vi "Main.vi"(8 "error in":errorcluster, 10 "User Events":T1, 11 "Message Queues in":T2) -> (0 "error out":errorcluster)   [LabVIEW 2020, in "MHL Templete.lvlib"]
doc: "This template is for the Queued Message Handler design pattern.\n\nThe Event Handling Loop generates messages based on user interface actions.\n\nThe Message Handling Loop processes messages generated by the Event Handling Loop, or by other messages. The messages are string values, so new messages can be added easily to the Message Cases case structure in the Message Handling Loop. Each message cluster can also provide an optional value for Message Data, which is a variant that can be converted to whatever message-specific data is required."
uses:
  MHL Templete.lvlib
  <vilib>/ErrorRing/Error Ring.xnode
  Type Definitions/Data.ctl
  support/Message Queue/Message Queue.lvlib
  support/User Event - Stop/User Event - Stop.lvlib
  <vilib>/Utility/error.llb/Error Cluster From Error Code.vi
  support/Message Queue/Message Cluster.ctl
  support/Message Queue/All Message Queues.ctl
  support/User Event - Stop/User Events.ctl
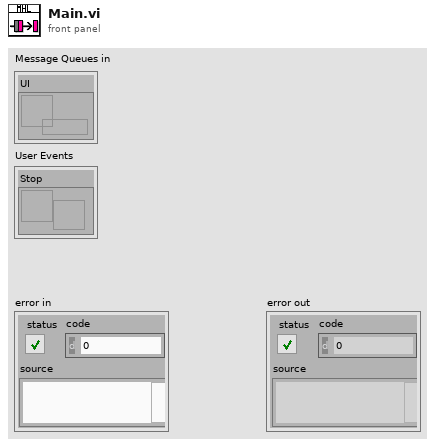
[diagram p1: front panel]
types:
  T1 = typedef "User Event - Stop.lvlib/User Events.ctl" = cluster{"Stop":refnum<user-event>}
  T2 = typedef "Message Queue.lvlib/All Message Queues.ctl" = cluster{"UI":refnum<queue>}
  T3 = typedef "MHL Templete.lvlib/Data.ctl" = cluster{"Boolean <Replace Me>":bool}
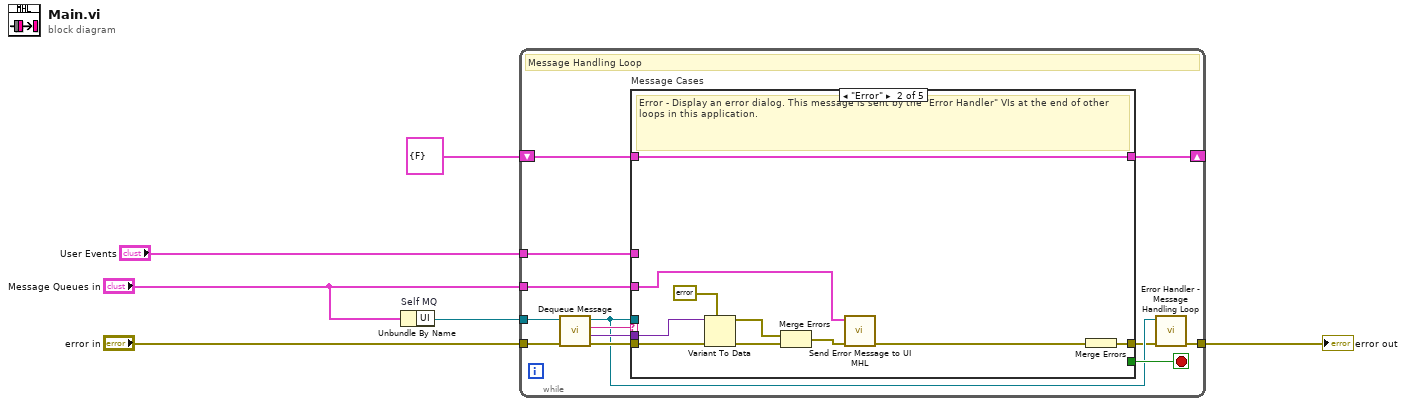
[diagram p0: block diagram]
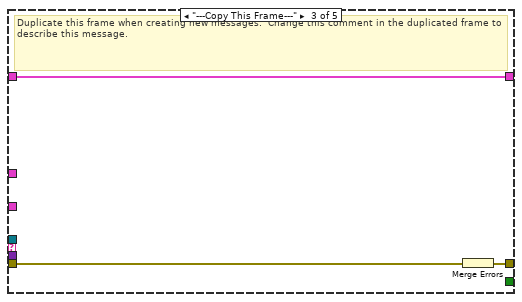
[diagram p3: hidden frame]
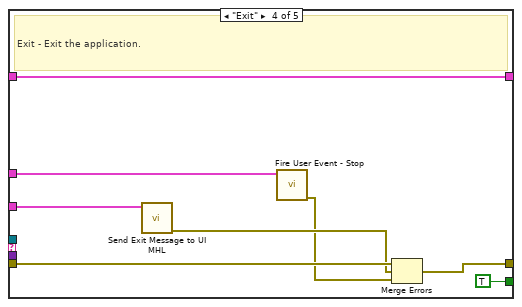
[diagram p4: hidden frame]
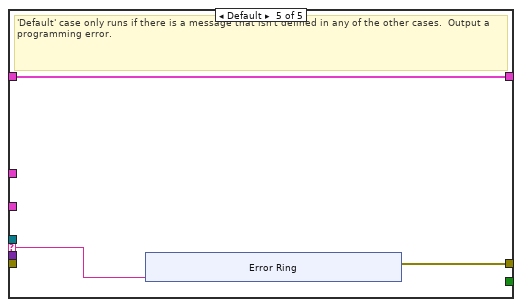
[diagram p5: hidden frame]
diagram:
  n1 = Unbundle By Name "Self MQ"("Message Queues in") -> ("UI"=w6:refnum<queue>)
  n2 = while {
    tunnel: w6 -> [w11]
    shift-right: [w18] -> _
    shift-left: T3 {"Boolean <Replace Me>"=FALSE} ("Data Cluster") -> [w19]
    tunnel: "User Events" -> [w16]
    tunnel: "error in" -> [w15]
    tunnel: [w9] -> w1
    tunnel: "Message Queues in" -> [w7]
    stop <- w17 stop-if-true
    # "Message Handling Loop"
    n3 = call "Dequeue Message.vi"("error in (no error)"=w15, "Message Queue"=w11) -> ("error out"=w14:errorcluster, "Message Data"=w12:variant, "Message"=w13:string, "dup Message Queue"=w10:refnum<queue>)  [unwired: 6 in]
    n4 = case "Message Cases" shown="\"Error\"" w13 {
      selector: w13 -> [_ _ _ _ w43]
      tunnel: w10 -> [_ _ _ _ _]
      tunnel: w14 -> [w21 w31 w34 w37 _]
      tunnel: [w21 w27 w32 w40 w44] -> w8
      tunnel: w19 -> [w20 w30 w33 w42 w45]
      tunnel: [w20 w30 w33 w42 w45] -> w18
      tunnel: [_ _ _ TRUE _] -> w17
      tunnel: w12 -> [_ w29 _ _ _]
      tunnel: w16 -> [_ _ _ w39 _]
      tunnel: w7 -> [_ w26 _ w38 _]
      frame "Initialize" {
        # "Initialize - All initialization work should take place in this message, since other loops can potentially enqueue messages that execute immediately after this one."
      }
      frame "Error" {
        # "Error - Display an error dialog. This message is sent by the \"Error Handler\" VIs at the end of other loops in this application."
        n5 = Variant To Data(error in=w31, type=errorcluster {"status"=FALSE, "code"=0, "source"=""} ("error constant"), Variant=w29) -> (data=w24:errorcluster, error out=w23:errorcluster)
        n6 = Merge Errors(w24, w23) -> (w22:errorcluster)
        n7 = call "Send Error Message to UI MHL.vi"("error in (no error)"=w22, "Message Queues"=w26) -> ("error out"=w25:errorcluster)  [unwired: 9 in]
        n8 = Merge Errors(w25) -> (w27:errorcluster)
      }
      frame "---Copy This Frame---" {
        # "Duplicate this frame when creating new messages.  Change this comment in the duplicated frame to describe this message."
        n9 = Merge Errors(w34) -> (w32:errorcluster)
      }
      frame "Exit" {
        # "Exit - Exit the application."
        n10 = call "Send Exit Message to UI MHL.vi"("Message Queues"=w38) -> ("error out"=w36:errorcluster)  [unwired: 10 in]
        n11 = call "Fire User Event - Stop.vi"("User Events"=w39) -> ("error out"=w35:errorcluster)  [unwired: 10 in]
        n12 = Merge Errors(w37, w36, w35) -> (w40:errorcluster)
      }
      frame Default {
        # "'Default' case only runs if there is a message that isn't defined in any of the other cases.  Output a programming error."
        n13 = xnode "Error Ring"("parameter 0"=w43) -> ("error out"=w44:errorcluster)
      }
    }
    n14 = call "Error Handler - Message Handling Loop.vi"("error in (no error)"=w8, "Message Queue"=w10) -> ("dup error in"=w9:errorcluster)  [unwired: 8 in, 1 out]
  }
  "error out" <- w1
